vi "Prog.vi"(8 "error in (no error) 2":errorcluster) -> (0 "error out":errorcluster, 2 "RESULT":bool, 3 "Result":string)   [LabVIEW 2021]
panel:
  out "standard error":string
  out "concatenated string 2":string
  out "standard output 2":string
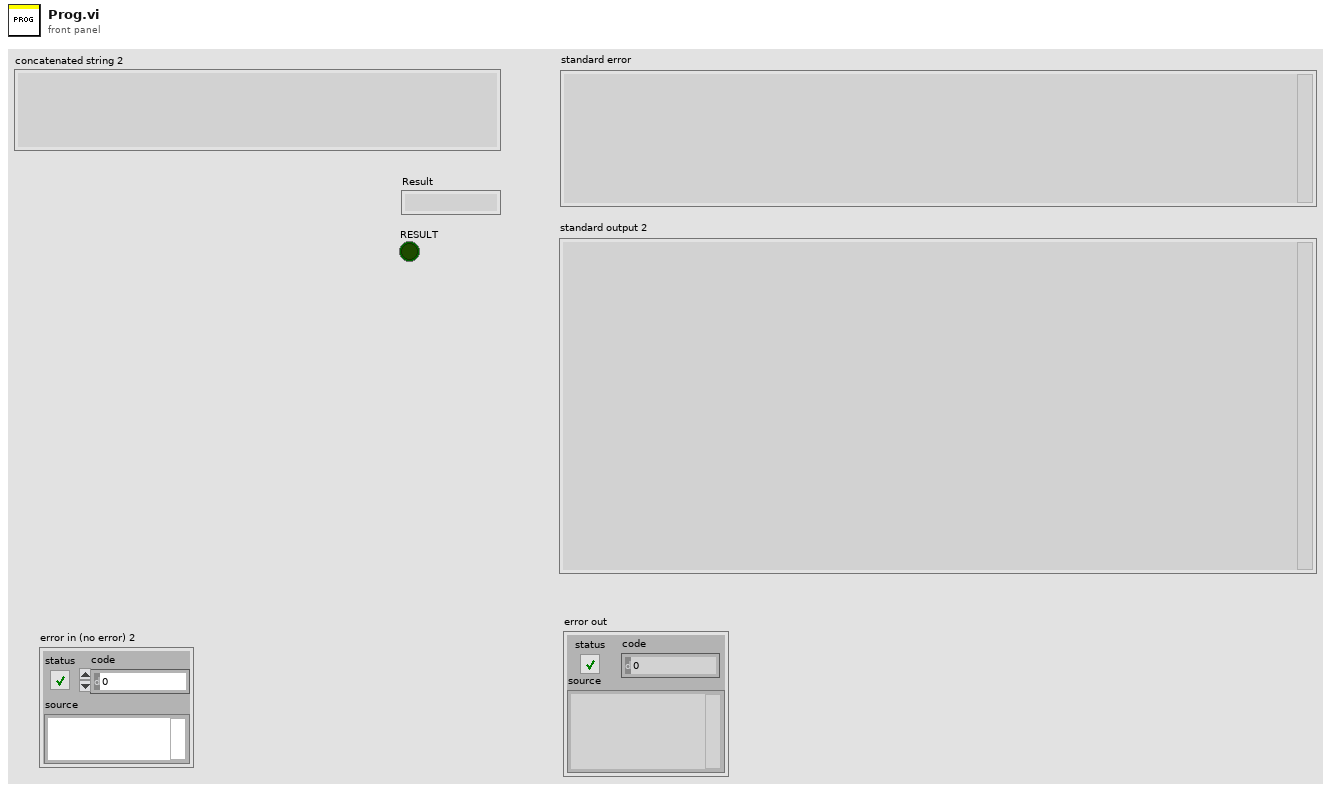
[diagram p1: front panel]
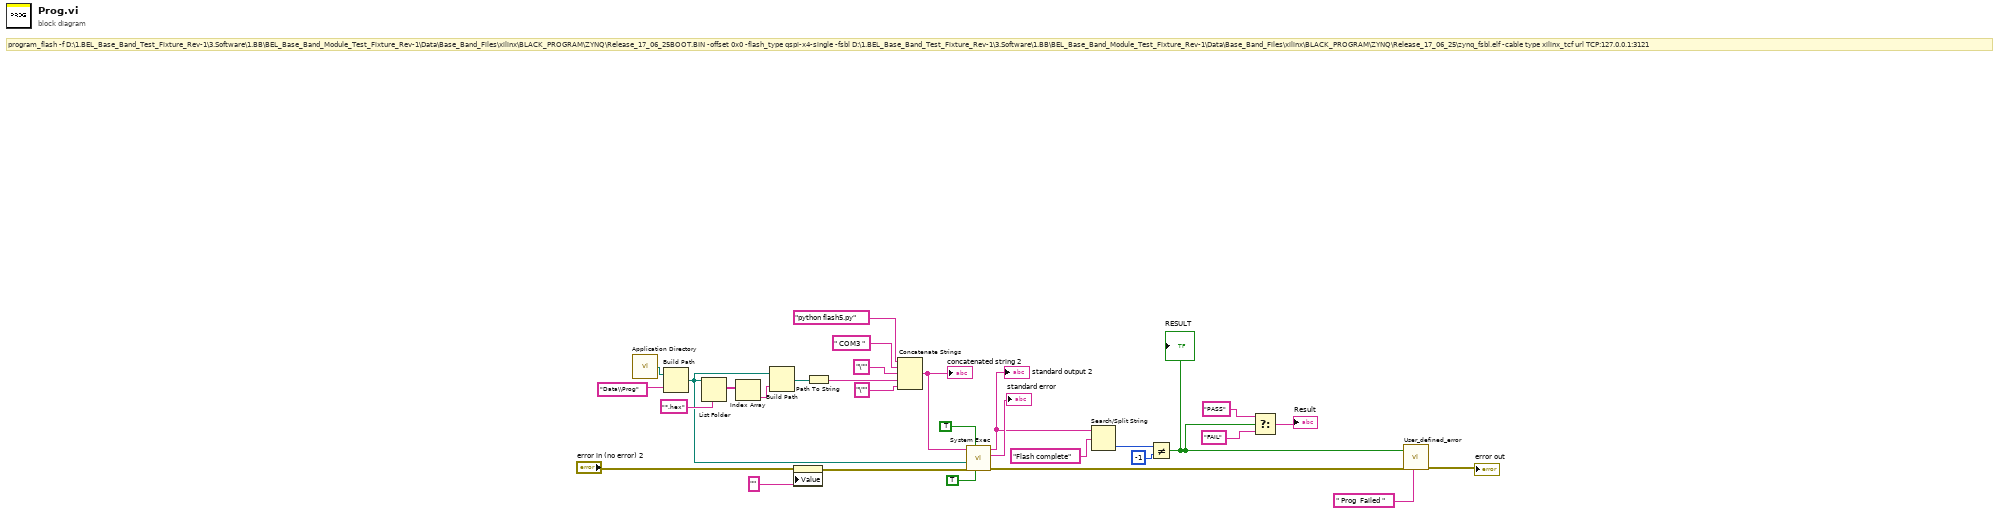
[diagram p0: block diagram]
diagram:
  # "program_flash -f D:\\1.BEL_Base_Band_Test_Fixture_Rev-1\\3.Software\\1.BB\\BEL_Base_Band_Module_Test_Fixture_Rev-1\\Data\\Base_Band_Files\\xilinx\\BLACK_PROGRAM\\ZYNQ\\Release_17_06_25BOOT.BIN -offset 0x0 -flash_type qspi-x4-single -fsbl D:\\1.BEL_Base_Band_Test_Fixture_Rev-1\\3.Software\\1.BB\\BEL_Base_Band_Module_Test_Fixture_Rev-1\\Data\\Base_Band_Files\\xilinx\\BLACK_PROGRAM\\ZYNQ\\Release_17_06_25\\zynq_fsbl.elf -cable type xilinx_tcf url TCP:127.0.0.1:3121"
  n1 = call <vilib>:"Application Directory.vi"() -> ("Application Directory"=w28:path)
  n2 = Build Path(base path=w28, name or relative path="Data\\Prog") -> (appended path=w15:path)
  n3 = List Folder(path=w15, pattern="*.hex") -> (filenames=w26:string[])  [unwired: 2 in, 3 out]
  n4 = Index Array(array=w26) -> (element=w24:string)  [unwired: 1 in]
  n5 = Build Path(base path=w15, name or relative path=w24) -> (appended path=w25:path)
  n6 = property on="standard output 2" class="Str"(error in="error in (no error) 2", "Value"="") -> (error out=w19:errorcluster)  [unwired: 1 in, 1 out]
  n7 = Path To String(path=w25) -> (string=w22:string)
  n8 = Concatenate Strings("python flash5.py", " COM3 " ("string"), "\"" ("string"), w22, "\"" ("string")) -> (w13:string)
  "concatenated string 2" <- w13
  n9 = call <vilib>:"System Exec.vi"("run minimized? (F)"=TRUE, "wait until completion? (T)"=TRUE, "error in (no error)"=w19, "working directory"=w15, "command line"=w13) -> ("error out"=w6:errorcluster, "standard error"=→"standard error":string, "standard output"=w1:string)  [unwired: 3 in, 1 out]
  "standard output 2" <- w1
  n10 = Search/Split String(string=w1, search string/char (-)="Flash complete") -> (offset of match=w11:i32)  [unwired: 1 in, 2 out]
  n11 = Not Equal?(x=w11, y=-1) -> (x != y?=w5:bool)
  "RESULT" <- w5
  n12 = Select(t="PASS", s=w5, f="FAIL") -> (s? t:f=→"Result":string)
  n13 = call "User_defined_error.vi"("Error Msg"=" Prog  Failed " ("source"), "error in"=w6, "Result"=w5) -> ("error Out"=→"error out":errorcluster)  [unwired: 8 in]
